vi "CSE routine - Call FuncVI.vi"(4 "CSE RefNum":T1, 5 "CE InstanceRef":T2, 6 "error code":i32, 9 "ParNum":i32) -> (0 "error code out":i32)   [LabVIEW 2021]
doc: "::: CalcExpress Toolkit :::\nCopyright (c) 2000-2026 Konstantin Shifershteyn. All rights reserved."
uses:
  cetypes.llb/CalcExpress Instance RefNum.ctl
  CSE Instance RefNum.ctl
  cersrc/celveng32.dll
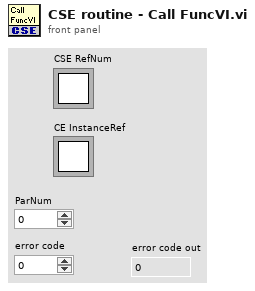
[diagram p1: front panel]
types:
  T1 = typedef "CSE Instance RefNum.ctl" = refnum<k1>
  T2 = typedef "CalcExpress Instance RefNum.ctl" = refnum<k1>
  T3 = cluster{"open to call":bool, "Enable FuncVI2":bool}
  T4 = typedef "CalcExpress Function Argument Info.ctl" = cluster{"type":u32, "str":string, "num":dbl}
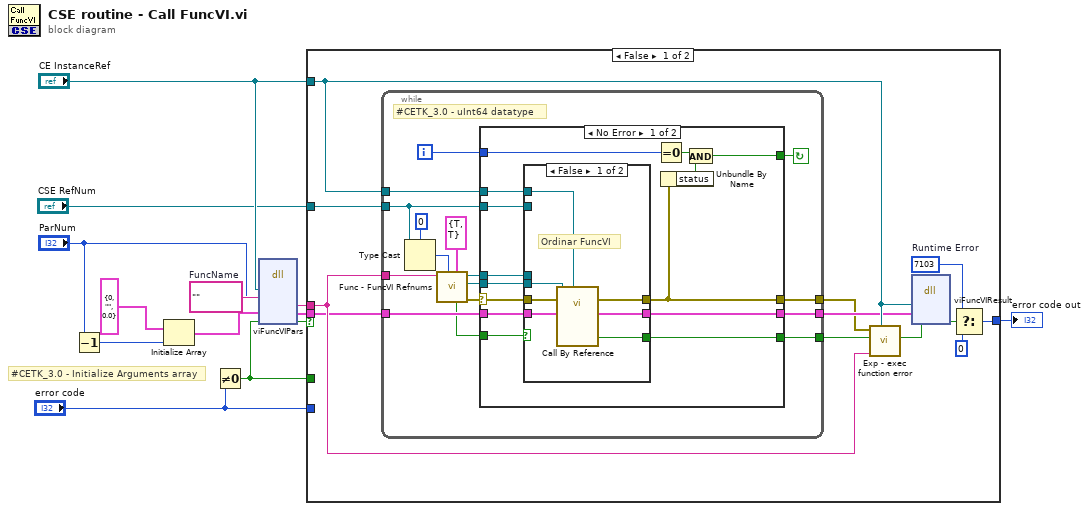
[diagram p0: block diagram]
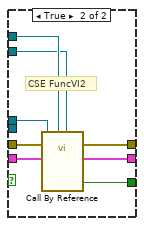
[diagram p2: hidden frame]
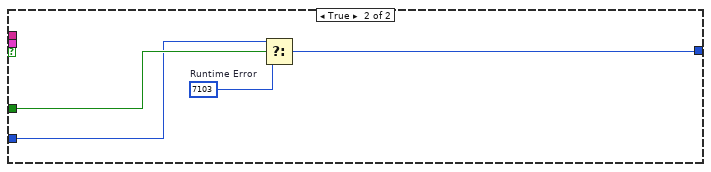
[diagram p4: hidden frame]
diagram:
  w12 = ""  # FuncName
  # "#CETK_3.0 - Initialize Arguments array"
  n1 = Decrement(x="ParNum") -> (x-1=w2:i32)
  n2 = Initialize Array(cluster{"type":u32, "str":string, "num":dbl} {"type"=0, "str"="", "num"=0.0} ("expr el out"), w2) -> (w4:cluster{"type":u32, "str":string, "num":dbl}[])
  n3 = Not Equal To 0?(x="error code") -> (x != 0?=w7:bool)
  n4 = dll-call lib="C:/LV Projects/CalcExpress 40 LV2021/vi.lib/addons/CalcExpress/cersrc/celveng*.dll" fn="viFuncVIPars"("iRef"="CE InstanceRef", "nPars"="ParNum", "FuncName"=w12, "ArgList"=w4, "erf"=w7) -> ("FuncName"=w9:string, "ArgList"=w10:cluster{"type":u32, "str":string, "num":dbl}[], "erf"=w11:bool)  [unwired: 6 in, 2 out]
  n5 = case shown="False" w11 {
    tunnel: "CE InstanceRef" -> [w21 _]
    tunnel: w9 -> [w20 _]
    tunnel: w10 -> [w19 _]
    tunnel: [w22 w72] -> w8
    tunnel: w7 -> [_ w75]
    tunnel: "error code" -> [_ w74]
    tunnel: "CSE RefNum" -> [w14 _]
    frame False {
      w18 = 7103  # Runtime Error
      n6 = while {
        tunnel: [w37] -> w15
        tunnel: w20 -> [w26]
        tunnel: [w39] -> w17
        tunnel: [w38] -> w16
        tunnel: w19 -> [w40]
        tunnel: w21 -> [w36]
        tunnel: w14 -> [w29]
        i -> [w32]
        stop <- w35 continue-if-true
        # "#CETK_3.0 - uInt64 datatype"
        n7 = Type Cast(type=u64 0, x=w29) -> (*(type *) &x=w28:u64)
        n8 = call "Func - FuncVI Refnums.vi"("Params"=T3 {"open to call"=TRUE, "Enable FuncVI2"=TRUE}, "Instance ID"=w28, "Func name"=w26) -> ("error out"=w33:errorcluster, "FuncVI RefNum out"=w34:refnum<vi>, "FuncVI2 RefNum out"=w41:refnum<vi>, "FuncVI2"=w31:bool)  [unwired: 4 in, 1 out]
        n9 = case shown="No Error" w33 {
          selector: w33 -> [w48 w71]
          tunnel: w41 -> [w55 _]
          tunnel: w40 -> [w54 _]
          tunnel: [w53 _] -> w39
          tunnel: [w52 _] -> w38
          tunnel: [w42 w71] -> w37
          tunnel: w36 -> [w51 _]
          tunnel: [w45 _] -> w35
          tunnel: w34 -> [w50 _]
          tunnel: w29 -> [w49 _]
          tunnel: w32 -> [w44 _]
          tunnel: w31 -> [w43 _]
          frame No Error {
            n10 = case shown="False" w43 {
              tunnel: w48 -> [w62 w68]
              tunnel: w55 -> [_ w64]
              tunnel: w54 -> [w61 w67]
              tunnel: [w60 w70] -> w53
              tunnel: [w59 w69] -> w52
              tunnel: [w58 w63] -> w42
              tunnel: w51 -> [w57 w66]
              tunnel: w50 -> [w56 _]
              tunnel: w49 -> [_ w65]
              frame False {
                # "Ordinar FuncVI"
                n11 = call-by-ref "Call By Reference"(reference=w56, error in=w62, "InstanceRef"=w57, "arg list"=w61) -> (error out=w58:errorcluster, "error out"=w59:bool, "result"=w60:T4)  [unwired: 6 in, 1 out]
              }
              frame True {
                # "CSE FuncVI2"
                n12 = call-by-ref "Call By Reference"(reference=w64, error in=w68, "CSE RefNum"=w65, "InstanceRef"=w66, "arg list"=w67) -> (error out=w63:errorcluster, "error out"=w69:bool, "result"=w70:T4)  [unwired: 5 in, 1 out]
              }
            }
            n13 = Equal To 0?(x=w44) -> (x = 0?=w47:bool)
            n14 = Unbundle By Name(w42) -> ("status"=w46:bool)
            n15 = And(x=w47, y=w46) -> (x .and. y?=w45:bool)
          }
          frame Error {
          }
        }
      }
      n16 = call "Exp - exec function error.vi"("CE InstanceRef"=w21, "func name"=w20, "CE error in"=w16, "error in"=w15) -> ("CE error out"=w25:bool)  [unwired: 5 in]
      n17 = dll-call lib="C:/LV Projects/CalcExpress 40 LV2021/vi.lib/addons/CalcExpress/cersrc/celveng*.dll" fn="viFuncVIResult"("iRef"=w21, "result"=w17, "erf"=w25) -> ("erf"=w24:bool)  [unwired: 6 in, 2 out]
      n18 = Select(t=w18, s=w24, f=0) -> (s? t:f=w22:i32)
    }
    frame True {
      w73 = 7103  # Runtime Error
      n19 = Select(t=w74, s=w75, f=w73) -> (s? t:f=w72:i32)
    }
  }
  "error code out" <- w8
